vi "CallTestSuiteMethod.vi"(8 "error in":errorcluster, 10 "method":T1, 11 "TestSuite in":refnum<class "TestSuite.lvclass">) -> (0 "error out":errorcluster, 2 "Test Method Error":errorcluster, 3 "TestSuite out":refnum<class "TestSuite.lvclass">)   [LabVIEW 2013, in "TestSuite.lvclass"]
uses:
  TestSuite.lvclass
  Method--enum.ctl
  TestSuite.lvclass/TestSuite.ctl
  JKI Reuse/Filter Error Codes (Scalar)__jki_lib_error_handling -- VI Tester.vi
  Libraries/VITesterUtilities.lvlib
panel:
  # "JKI VI Tester for LabVIEW\nhttp://jkisoft.com/vi-tester\nCopyright (C) 2007-2009, JKI <info@jkisoft.com>\nALL RIGHTS RESERVED"
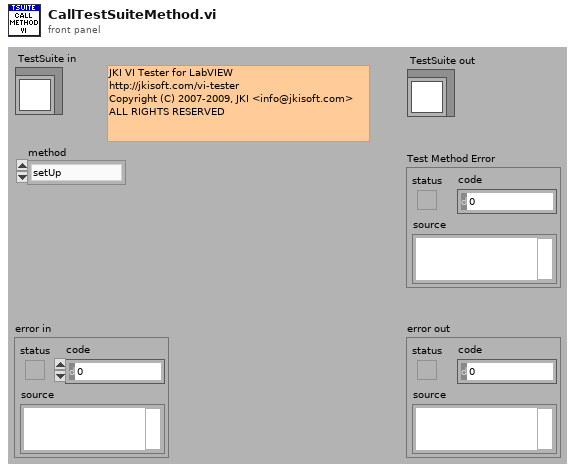
[diagram p1: front panel]
types:
  T1 = typedef "TestSuite.lvclass/Method--enum.ctl" = enum16{"setUp", "tearDown"}
  T2 = enum32{"Bad", "Idle", "Run top level", "Running"}
  T3 = cluster{"name":string, "type desc":i16[], "flat data":string}
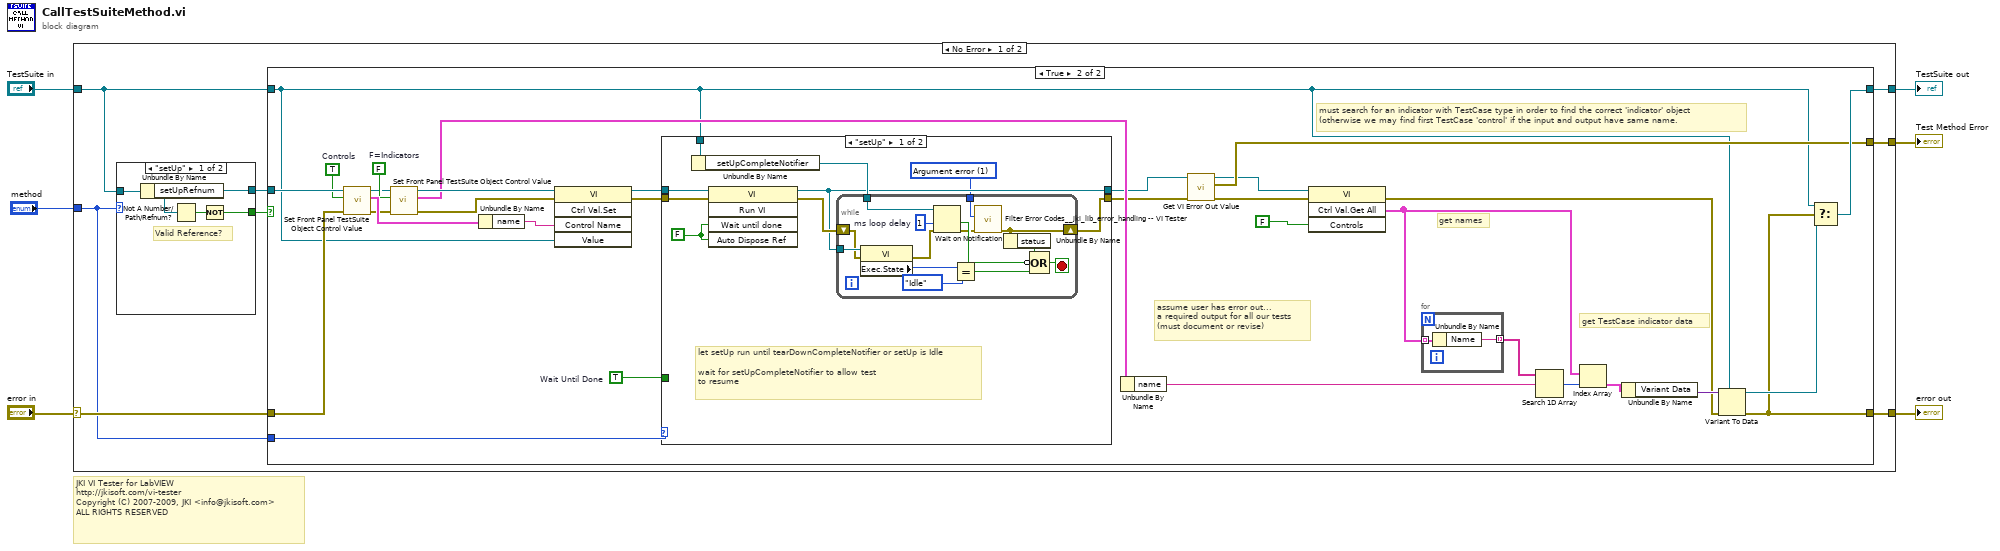
[diagram p0: block diagram]
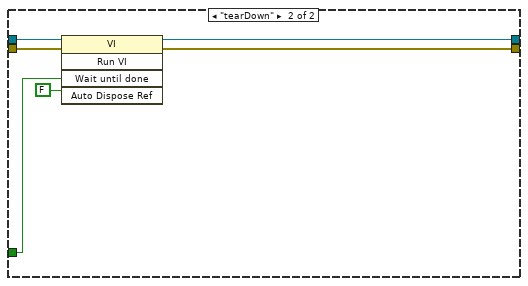
[diagram p3: hidden frame]
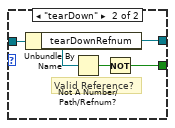
[diagram p4: hidden frame]
diagram:
  # "JKI VI Tester for LabVIEW\nhttp://jkisoft.com/vi-tester\nCopyright (C) 2007-2009, JKI <info@jkisoft.com>\nALL RIGHTS RESERVED"
  n1 = case shown="No Error" "error in" {
    selector: "error in" -> [w9 w89]
    tunnel: [w14 w88] -> w2
    tunnel: [w13 _] -> w3
    tunnel: [w12 w89] -> w4
    tunnel: "TestSuite in" -> [w11 w88]
    tunnel: "method" -> [w7 _]
    frame No Error {
      n2 = case shown="\"setUp\"" w7 {
        tunnel: w11 -> [w83 w87]
        tunnel: [w82 w86] -> w10
        tunnel: [w80 w84] -> w8
        frame "setUp" {
          # "Valid Reference?"
          n3 = Unbundle By Name(w83) -> ("setUpRefnum"=w82:refnum<vi>)
          n4 = Not A Number/Path/Refnum?(number/path/refnum=w82) -> (NaN/Path/Refnum?=w81:bool)
          n5 = Not(x=w81) -> (.not. x?=w80:bool)
        }
        frame "tearDown" {
          # "Valid Reference?"
          n6 = Unbundle By Name(w87) -> ("tearDownRefnum"=w86:refnum<vi>)
          n7 = Not A Number/Path/Refnum?(number/path/refnum=w86) -> (NaN/Path/Refnum?=w85:bool)
          n8 = Not(x=w85) -> (.not. x?=w84:bool)
        }
      }
      n9 = case shown="True" w8 {
        tunnel: [w16 w48] -> w14
        tunnel: [_ w19] -> w13
        tunnel: [w15 w27] -> w12
        tunnel: w11 -> [w16 w17]
        tunnel: w10 -> [_ w45]
        tunnel: w9 -> [w15 w37]
        tunnel: w7 -> [_ w35]
        frame False {
        }
        frame True {
          w34 = TRUE  # Wait Until Done
          w41 = FALSE  # F=Indicators
          w44 = TRUE  # Controls
          # "get TestCase indicator data"
          # "get names"
          # "must search for an indicator with TestCase type in order to find the correct 'indicator' object\n(otherwise we may find first TestCase 'control' if the input and output have same name."
          # "assume user has error out...\na required output for all our tests\n(must document or revise)"
          n10 = call "Set Front Panel TestSuite Object Control Value.vi"("error in"=w37, "Control (F: Indicator)"=w44, "vi reference"=w45) -> ("error out"=w40:errorcluster, "Control Value"=w43:T3, "dup vi reference"=w39:refnum<vi>)  [unwired: 5 in, 1 out]
          n11 = call "Set Front Panel TestSuite Object Control Value.vi"("error in"=w40, "Control (F: Indicator)"=w41, "vi reference"=w39) -> ("error out"=w36:errorcluster, "Control Value"=w26:T3, "dup vi reference"=w38:refnum<vi>)  [unwired: 5 in, 1 out]
          n12 = Unbundle By Name(w43) -> ("name"=w42:string)
          n13 = invoke class="VI" method="Ctrl Val.Set"(reference=w38, error in=w36, "Control Name"=w42, "Value"=w17) -> (reference out=w47:refnum<vi>, error out=w46:errorcluster)  [unwired: 1 in, 3 out]
          n14 = case shown="\"setUp\"" w35 {
            tunnel: w47 -> [w59 w79]
            tunnel: w46 -> [w58 w78]
            tunnel: [w52 w77] -> w22
            tunnel: [w53 w76] -> w21
            tunnel: w34 -> [_ w74]
            tunnel: w17 -> [w56 _]
            frame "setUp" {
              w51 = 1 items=["No error", "Argument error", "Memory is full", "Out of zone", "End of file", "File already open", "Generic file I/O error", "File not found", "File permission error", "Disk is full", "Duplicate path", "Too many files open", "System feature not enabled", "Resource file not found", "Cannot add resource", "Resource not found", "Image not found", "Image memory error", "Pen does not exist", "Config type invalid", "Config token not found", "Config parse error", "Config memory error", "Bad external code format", "Bad external code offset", "External code not present", "Null window", "Destroy window error", "Null menu", "Print aborted", "Bad print record", "Print driver error", "Windows error during printing", "Memory error during printing", "Print dialog error", "Generic print error", "Invalid device refnum", "Device not found", "Device parameter error", "Device unit error", "Cannot open device", "Device call aborted", "Generic error", "Cancelled by user", "Object ID too low", "Object ID too high", "Object not in heap", "Unknown heap", "Unknown object (invalid DefProc)", "Unknown object (DefProc not in table)", "Message out of range", "Invalid (null) method", "Unknown message", "Manager call not supported", "Bad address", "Network operation in progress", "Network operation timed out", "Connection is busy", "Network attribute not supported", "Network error", "Address in use", "System out of memory", "Connection aborted", "Connection refused", "Not connected", "Already connected", "Connection closed", "Initialization error (interapplication manager)", "Bad occurrence", "Wait on unbound occurrence handler", "Occurrence queue overflow", "Datalog type conflict", "Unused", "Unrecognized type (interapplication manager)", "Memory corrupt", "Failed to make temporary DLL", "Old CIN version", "Drag socket not found", "Failed to load drop-object", "Failed to register OLE object", "Failed to release OLE object", "Format specifier type mismatch", "Unknown format specifier", "Too few format specifiers", "Too many format specifiers", "Scan failed", "Newer CIN version", "Error converting to variant", "Runtime menu error", "Password tampered", "Variant attribute not found", "Incompatible variant data type", "Event data is not available", "Event Store is not present", "Occurrence is not found", "Event Queue is not created", "Event info is not available", "Refnum passed is NULL", "Error retrieving Class GUID", "Error retrieving CoClass GUID", "Error retrieving TypeLib GUID.", "Bad built application magic bytes.", "Specific driver is different from the specific driver associated with the Logical Name.", "There is no session opened to the class driver.", "Max Error", "MAX - Error with config objects", "MAX - Error loading configuration", "MAX - Group not supported"]
              w57 = FALSE ("Auto Dispose Reference")
              # "let setUp run until tearDownCompleteNotifier or setUp is Idle\n\nwait for setUpCompleteNotifier to allow test\nto resume"
              n15 = Unbundle By Name(w56) -> ("setUpCompleteNotifier"=w55:refnum<notifier>)
              n16 = invoke class="VI" method="Run VI"(reference=w59, error in=w58, "Wait until done"=w57, "Auto Dispose Ref"=w57) -> (reference out=w52:refnum<vi>, error out=w54:errorcluster)  [unwired: 1 in, 3 out]
              n17 = while {
                tunnel: w55 -> [w73]
                tunnel: w52 -> [w71]
                shift-right: [w61] -> w53
                shift-left: w54 -> [w70]
                tunnel: w51 -> [w60]
                stop <- w63 stop-if-true
                w72 = 1  # ms loop delay
                n18 = property class="VI"(reference=w71, error in=w70) -> (error out=w69:errorcluster, "Exec.State"=w68:T2)  [unwired: 1 out]
                n19 = Wait on Notification(notifier=w73, timeout in ms (-1)=w72, error in (no error)=w69) -> (timed out?=w65:bool, error out=w62:errorcluster)  [unwired: 1 in, 2 out]
                n20 = Equal?(x=w68, y=T2."Idle") -> (x = y?=w66:bool)
                n21 = call-poly "Filter Error Codes__jki_lib_error_handling -- VI Tester.vi"("error in"=w62, "error code to filter"=w60) -> ("error out"=w61:errorcluster)  [unwired: 7 in, 2 out]
                n22 = Unbundle By Name(w61) -> ("status"=w64:bool)
                n23 = Compound Arithmetic op=OR(w64, invert w65, w66) -> (w63:bool)
              }
            }
            frame "tearDown" {
              n24 = invoke class="VI" method="Run VI"(reference=w79, error in=w78, "Wait until done"=w74, "Auto Dispose Ref"=FALSE ("Auto Dispose Reference")) -> (reference out=w77:refnum<vi>, error out=w76:errorcluster)  [unwired: 1 in, 3 out]
            }
          }
          n25 = Unbundle By Name(w26) -> ("name"=w23:string)
          n26 = call "Get VI Error Out Value.vi"("error in"=w21, "vi reference in"=w22) -> ("error out"=w20:errorcluster, "vi error out"=w19:errorcluster, "dup vi reference"=w18:refnum<vi>)  [unwired: 7 in]
          n27 = invoke class="VI" method="Ctrl Val.Get All"(reference=w18, error in=w20, "Controls"=FALSE) -> (error out=w28:errorcluster, "Get All Control Values Variant"=w25:cluster{"Name":string, "Variant Data":variant}[])  [unwired: 1 in, 2 out]
          n28 = for {
            tunnel: w25 -> [w50] mode=indexing
            tunnel: [w49] -> w24 mode=indexing
            n29 = Unbundle By Name(w50) -> ("Name"=w49:string)
          }
          n30 = Search 1D Array(1D array=w24, element=w23) -> (index of element=w32:i32)  [unwired: 1 in]
          n31 = Index Array(array=w25, index=w32) -> (element=w31:cluster{"Name":string, "Variant Data":variant})
          n32 = Unbundle By Name(w31) -> ("Variant Data"=w30:variant)
          n33 = Variant To Data(error in=w28, type=w17, Variant=w30) -> (data=w29:refnum<class "TestSuite.lvclass">, error out=w27:errorcluster)
          n34 = Select(t=w17, s=w27, f=w29) -> (s? t:f=w48:refnum<class "TestSuite.lvclass">)
        }
      }
    }
    frame Error {
    }
  }
  "error out" <- w4
  "Test Method Error" <- w3
  "TestSuite out" <- w2
